vi "Create FIFO Config Extended.vi"(11 "New FIFO Config":T1) -> (3 "Flattened FIFO Config":u8[](array[numeric]))   [LabVIEW 2021, in "ChannelCommon.lvlib"]
doc: "This will create the flattened FIFO configuration used to override the default settings when creating a new FIFO reader or writer. If no configuration is provided the default for that FIFO type will be used. \n\nThis configuration is also used on tag writers with variable length input such as string tags. For tags only the Max Bytes/Msg element is used and other fields are ignored. \n\nIf additional custom data is needed by the FIFO type this can be appended to the end of the flattened data. This custom data will be FIFO specific and is not commonly used."
uses:
  typedef/New FIFO Config.ctl
  typedef/FIFO Flags.ctl
  typedef/FIFO Config Extended.ctl
  ChannelCommon.lvlib
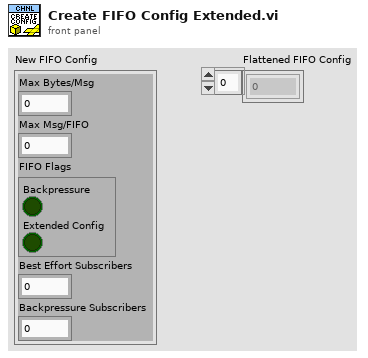
[diagram p1: front panel]
types:
  T1 = typedef "ChannelCommon.lvlib/New FIFO Config.ctl" = cluster{"Max Bytes/Msg":u64, "Max Msg/FIFO":u64, "FIFO Flags":T2, "Best Effort Subscribers":u32, "Backpressure Subscribers":u32}
  T2 = typedef "ChannelCommon.lvlib/FIFO Flags.ctl" = cluster{"Backpressure":bool, "Extended Config":bool}
  T3 = typedef "ChannelCommon.lvlib/FIFO Config Extended.ctl" = cluster{"Max Bytes/Msg":u64, "Max Msg/FIFO":u64, "Flags":u64, "Best Effort Subscribers":u32, "Backpressure Subscribers":u32, "Custom Data":u8[]}
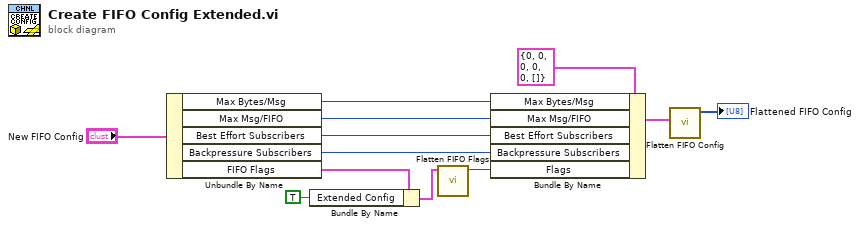
[diagram p0: block diagram]
diagram:
  n1 = Unbundle By Name("New FIFO Config") -> ("Max Bytes/Msg"=w11:u64, "Max Msg/FIFO"=w10:u64, "Best Effort Subscribers"=w1:u32, "Backpressure Subscribers"=w2:u32, "FIFO Flags"=w5:T2)
  n2 = Bundle By Name(cluster=w5, "Extended Config"=TRUE) -> (w3:T2)
  n3 = call "Flatten FIFO Flags.vi"("Flags"=w3) -> ("FIFO Flags"=w6:u64)  [unwired: 10 in]
  n4 = Bundle By Name(cluster=T3 {"Max Bytes/Msg"=0, "Max Msg/FIFO"=0, "Flags"=0, "Best Effort Subscribers"=0, "Backpressure Subscribers"=0, "Custom Data"=[]} ("FIFO Config"), "Max Bytes/Msg"=w11, "Max Msg/FIFO"=w10, "Best Effort Subscribers"=w1, "Backpressure Subscribers"=w2, "Flags"=w6) -> (w7:T3)
  n5 = call "Flatten FIFO Config.vi"("FIFO Config Extended in"=w7) -> ("Flattened FIFO Config"=→"Flattened FIFO Config":u8[])  [unwired: 10 in]
